vi "[ce] Curve Length.vi"(6 "parameters":cluster{"name":string, "value":dbl}[](array[cluster]) {"value" format="%.2f"}, 7 "# points":u32=200, 8 "error in":errorcluster, 9 "formula info":cluster{"formula":string, "x-variable":string}={"formula"="", "x-variable"="x"}, 10 "end":dbl=1.0 format="%.2f", 11 "start":dbl format="%.2f") -> (0 "error out":errorcluster, 1 "ticks":u32, 2 "Curve Length":dbl[](array[numeric]) format="%.2f", 3 "X Values":dbl[](array[numeric]) format="%.2f")   [LabVIEW 2021]
doc: "Calculates the curve length of a 1D function between start and end points. In addition, the VI allows specifying additional parameters and evaluating them in formula.\n\n::: CalcExpress Toolkit :::\nCopyright (c) 2000-2026 Konstantin Shifershteyn. All rights reserved."
panel:
  # "Example 1:\n---------------\nformula info:\n  formula: sin(t)\n  x-variable: t\nparameters:  empty array\n\nExample 2:\n---------------\nformula info:\n  formula: a*sin(x)*exp(-x/b)\n  x-variable: x\nparameters: (a,1), (b,2)"
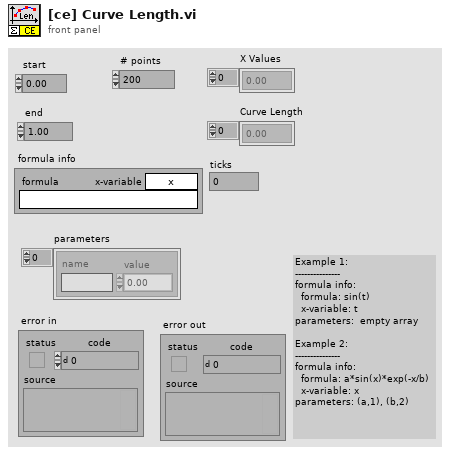
[diagram p1: front panel]
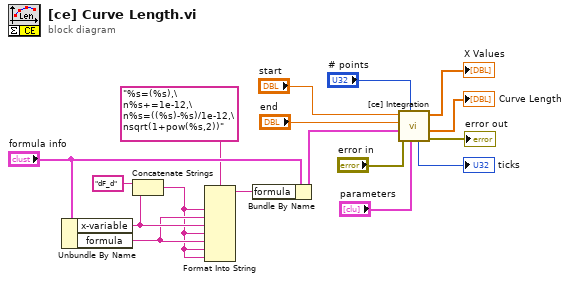
[diagram p0: block diagram]
diagram:
  n1 = Unbundle By Name("formula info") -> ("x-variable"=w16:string, "formula"=w15:string)
  n2 = Concatenate Strings("dF_d" ("Substring"), w16) -> (w1:string)
  n3 = Format Into String(format string="%s=(%s),\n%s+=1e-12,\n%s=((%s)-%s)/1e-12,\nsqrt(1+pow(%s,2))" ("Format String"), w1, w15, w16, w1, w15, w1, w1) -> (resulting string=w3:string)  [unwired: 2 in, 1 out]
  n4 = Bundle By Name(cluster="formula info", "formula"=w3) -> (w13:cluster{"formula":string, "x-variable":string})
  n5 = call "[ce] Integration.vi"("parameters"="parameters", "# points"="# points", "error in"="error in", "formula info"=w13, "end"="end", "start"="start") -> ("error out"=→"error out":errorcluster, "Integral of Y"=→"Curve Length":dbl[], "X Values"=→"X Values":dbl[], "ticks"=→"ticks":u32)  [unwired: 1 in, 1 out]
